vi "Accumulate N.vi"(0 "N":i32=5) -> (1 "Sum":i32, 2 "Count":i32)   [LabVIEW 2026]
doc: "Round20 multi-VI demo subVI (P6): a While Loop with two shift registers accumulating Sum = 1+2+...+N and Count = N over N iterations (element = iteration index + 1). Panel: N in (conIdx0, required), Sum out (conIdx1, recommended), Count out (conIdx2, recommended). Same loop dialect as the proven Accumulator (LV020): SR seeds stay on the root diagram, loop-internal constants enter via tunnels, stop condition is Greater Or Equal? feeding the Condition terminal."
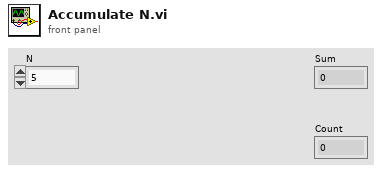
[diagram p1: front panel]
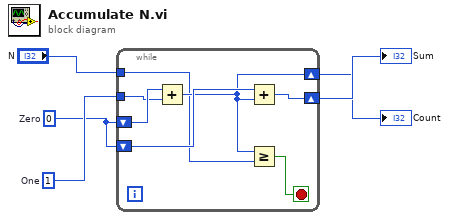
[diagram p0: block diagram]
diagram:
  w3 = 1  # One
  w2 = 0  # Zero
  n1 = while {
    tunnel: "N" -> [w6]
    tunnel: w3 -> [w7]
    shift-right: [w9] -> w4
    shift-left: w2 -> [w8]
    shift-right: [w11] -> w5
    shift-left: w2 -> [w10]
    stop <- w12 stop-if-true
    n2 = Add(x=w8, y=w7) -> (x+y=w9:i32)
    n3 = Add(x=w10, y=w9) -> (x+y=w11:i32)
    n4 = Greater Or Equal?(x=w9, y=w6) -> (x >= y?=w12:bool)
  }
  "Sum" <- w5
  "Count" <- w4
